vi "RichToFlatlv_python_grpc_webui_demo_v1_ChamberStatus.vi"(5 "OutputClusterType":T1, 11 "InputCluster":T3) -> (3 "OutputCluster":T1)   [LabVIEW 2020, in "thermal-chamber-controller_server.lvlib"]
uses:
  thermal-chamber-controller_server.lvlib
  lv_python_grpc_webui_demo_v1_ChamberStatus.ctl
  lv_python_grpc_webui_demo_v1_HeaterState.ctl
  lv_python_grpc_webui_demo_v1_ChamberStatus_Flat.ctl
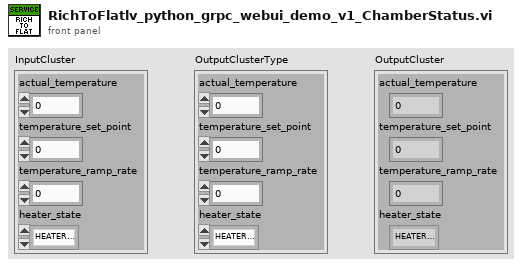
[diagram p1: front panel]
types:
  T1 = typedef "thermal-chamber-controller_server.lvlib/lv_python_grpc_webui_demo_v1_ChamberStatus_Flat.ctl" = cluster{"actual_temperature":dbl, "temperature_set_point":dbl, "temperature_ramp_rate":dbl, "heater_state":T2}
  T2 = typedef "thermal-chamber-controller_server.lvlib/lv_python_grpc_webui_demo_v1_HeaterState.ctl" = enum32{"HEATER_ENABLED", "HEATER_DISABLED"}
  T3 = typedef "thermal-chamber-controller_server.lvlib/lv_python_grpc_webui_demo_v1_ChamberStatus.ctl" = cluster{"actual_temperature":dbl, "temperature_set_point":dbl, "temperature_ramp_rate":dbl, "heater_state":T2}
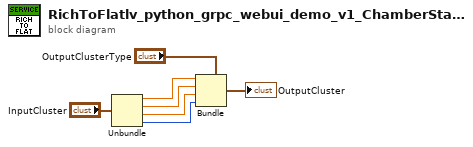
[diagram p0: block diagram]
diagram:
  n1 = Unbundle "Unbundle"("InputCluster") -> ("actual_temperature"=w4:dbl, "temperature_set_point"=w3:dbl, "temperature_ramp_rate"=w2:dbl, "heater_state"=w1:T2)
  n2 = Bundle "Bundle"(cluster="OutputClusterType", "actual_temperature"=w4, "temperature_set_point"=w3, "temperature_ramp_rate"=w2, "heater_state"=w1) -> (→"OutputCluster":T1)
